vi "Native_GetGlobalControlName.vi"() -> ()   [LabVIEW 2024]
panel:
  out "error out":errorcluster caption="错误输出"
  out "control_name":string
  in  "global_id":u32
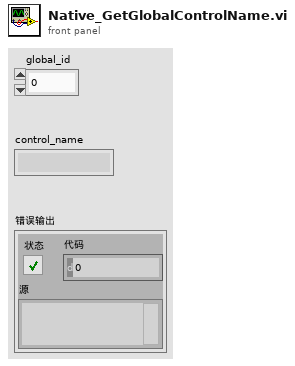
[diagram p1: front panel]
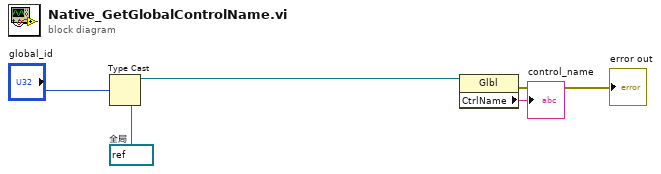
[diagram p0: block diagram]
diagram:
  w4 = refnum<vi> refnum  # 全局
  n1 = Type Cast ("强制类型转换")(type=w4, x="global_id") -> (*(type *) &x=w3:refnum<vi>)
  n2 = property on="属性节点" class="Glbl"(reference=w3) -> (error out=→"error out":errorcluster, "CtrlName"=→"control_name":string)  [unwired: 1 in, 1 out]
